vi "Generate SQL.vi"(8 "error in (no error)":errorcluster, 11 "SQLite Connection in":refnum<class "Connection.lvclass">) -> (0 "error out":errorcluster, 2 ".sql File Path":path, 3 "SQLite Connection out":refnum<class "Connection.lvclass">)   [LabVIEW 2024, in "DBMigrations.lvlib"]
doc: "Output schema and data to .sql file in same location as database."
uses:
  DBMigrations.lvlib
  <vilib>/drjdpowell/SQLite Library/SQL Connection/Connection.lvclass
  <vilib>/drjdpowell/SQLite Library/SQL Connection/Connection.lvclass/Connection.ctl
  <vilib>/Utility/error.llb/Trim Whitespace One-Sided.vi
  <vilib>/drjdpowell/SQLite Library/SQL Connection/Execute SQL (1D String).vi
  <vilib>/drjdpowell/SQLite Library/SQL Connection/Execute SQL.vi
  <vilib>/drjdpowell/SQLite Library/SQLite.lvlib
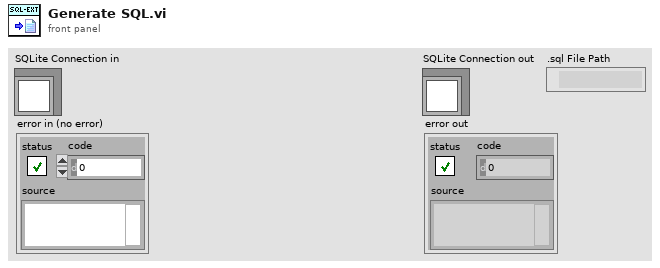
[diagram p1: front panel]
types:
  T1 = enum16{"open", "replace", "create", "open or create", "replace or create", "replace or create with confirmation"}
  T2 = typedef "DB-Migrations.lvlib/Schema.ctl" = cluster{"table name":string, "table info":cluster{"cid":string, "name":string, "type":string, "notnull":string, "dflt_value":string, "pk":string, "unique":string}[]}[]
  T3 = cluster{"cid":string, "name":string, "type":string, "notnull":string, "dflt_value":string, "pk":string, "unique":string}[]
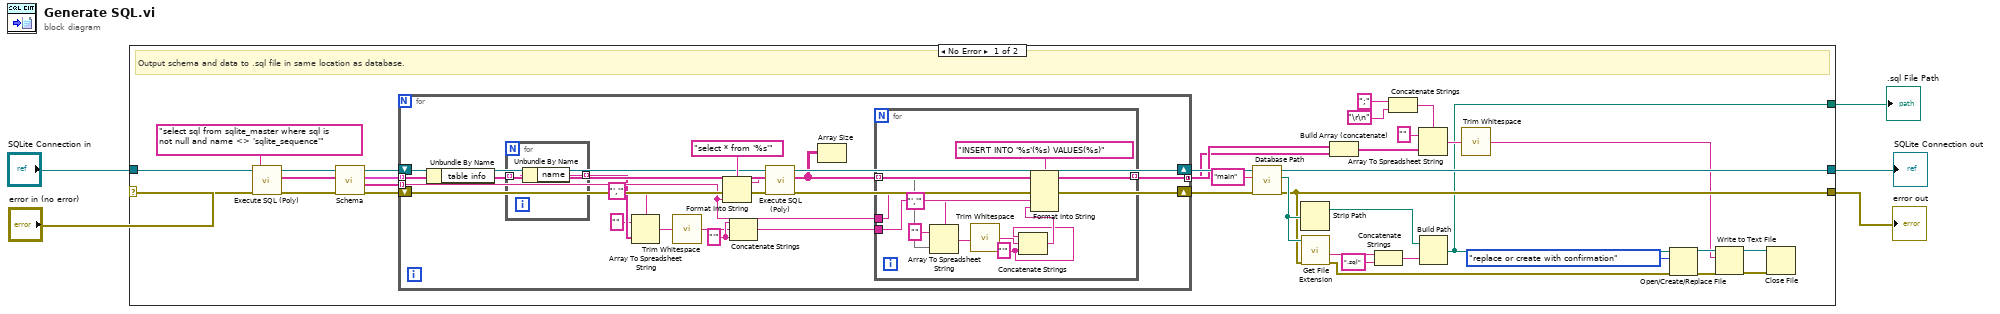
[diagram p0: block diagram]
diagram:
  n1 = case shown="No Error" "error in (no error)" {
    selector: "error in (no error)" -> [w22 w73]
    tunnel: "SQLite Connection in" -> [w40 w74]
    tunnel: [w37 w74] -> w4
    tunnel: [w29 w73] -> w3
    tunnel: [w21 _] -> w1
    frame No Error {
      # "Output schema and data to .sql file in same location as database."
      n2 = call-poly <vilib>:"Execute SQL (Poly).vi"("error in (no error)"=w22, "SQL"="select sql from sqlite_master where sql is not null and name <> 'sqlite_sequence'", "SQLite Connection in"=w40) -> ("error out"=w16:errorcluster, "Result Set"=w9:string[], "SQLite Connection"=w17:refnum<class "Connection.lvclass">)  [unwired: 5 in, 1 out]
      n3 = call "Schema.vi"("error in (no error)"=w16, "SQLite Connection In"=w17) -> ("error out"=w14:errorcluster, "Table Names"=w15:string[], "Schema"=w10:T2, "SQLite Connection Out"=w13:refnum<class "Connection.lvclass">)  [unwired: 6 in]
      n4 = for {
        tunnel: w15 -> [w49] mode=indexing
        shift-right: [w55] -> w12
        shift-left: w14 -> [w56]
        shift-right: [w53] -> w11
        shift-left: w13 -> [w54]
        tunnel: w10 -> [w51] mode=indexing
        tunnel: [w42] -> w7 mode=concatenating
        w43 = "'" ("string")
        n5 = Unbundle By Name(w51) -> ("table info"=w50:T3)
        n6 = for {
          tunnel: w50 -> [w61] mode=indexing
          tunnel: [w60] -> w48 mode=indexing
          n7 = Unbundle By Name(w61) -> ("name"=w60:string)
        }
        n8 = Array To Spreadsheet String(delimiter (Tab)="','", array=w48, 3:"" ("format string")) -> (spreadsheet string=w45:string)
        n9 = call <vilib>:"Trim Whitespace.vi"("string"=w45) -> ("trimmed string"=w41:string)  [unwired: 1 in]
        n10 = Format Into String(format string="select * from '%s'" ("SQL"), error in=w56, w49) -> (resulting string=w57:string, error out=w58:errorcluster)  [unwired: 1 in]
        n11 = Concatenate Strings(w43, w41, w43) -> (w44:string)
        n12 = call-poly <vilib>:"Execute SQL (Poly).vi"("error in (no error)"=w58, "SQL"=w57, "SQLite Connection in"=w54) -> ("error out"=w55:errorcluster, "Result Set"=w52:string[][], "SQLite Connection"=w53:refnum<class "Connection.lvclass">)  [unwired: 5 in, 1 out]
        n13 = Array Size(array=w52) -> ()  [unwired: 1 out]
        n14 = for {
          tunnel: w52 -> [w69] mode=indexing
          tunnel: w49 -> [w71]
          tunnel: w44 -> [w70]
          tunnel: [w63] -> w42 mode=indexing
          w64 = "'" ("string")
          n15 = Array To Spreadsheet String(delimiter (Tab)="','", array=w69, 3:"" ("format string")) -> (spreadsheet string=w65:string)
          n16 = call <vilib>:"Trim Whitespace.vi"("string"=w65) -> ("trimmed string"=w62:string)  [unwired: 1 in]
          n17 = Concatenate Strings(w64, w62, w64) -> (w66:string)
          n18 = Format Into String(format string="INSERT INTO '%s'(%s) VALUES(%s)" ("SQL"), w71, w70, w66) -> (resulting string=w63:string)  [unwired: 2 in, 1 out]
        }
      }
      n19 = call <vilib>:"Database Path.vi"("error in (no error)"=w12, "Database Name (\"main\")"="main" ("Database Name (\"main\")"), "SQLite Connection in"=w11) -> ("error out"=w29:errorcluster, "Path to Database"=w35:path, "SQLite Connection"=w37:refnum<class "Connection.lvclass">)  [unwired: 6 in]
      n20 = Strip Path(path=w35) -> (stripped path=w36:path)  [unwired: 1 out]
      n21 = call <vilib>:"Get File Extension.vi"("error in (no error)"=w29, "file"=w35) -> ("error out"=w30:errorcluster, "filename without extension"=w34:string)  [unwired: 5 in, 3 out]
      n22 = Build Array (concatenate)(w9, w7) -> (w8:string[])
      n23 = Concatenate Strings(w34, ".sql" ("string")) -> (w32:string)
      n24 = Concatenate Strings(";" ("delimiter (Tab)"), "\r\n") -> (w18:string)
      n25 = Array To Spreadsheet String(delimiter (Tab)=w18, array=w8, 3:"" ("format string")) -> (spreadsheet string=w25:string)
      n26 = Build Path(base path=w36, name or relative path=w32) -> (appended path=w21:path)
      n27 = call <vilib>:"Trim Whitespace.vi"("string"=w25) -> ("trimmed string"=w6:string)  [unwired: 1 in]
      n28 = Open/Create/Replace File(file path (use dialog)=w21, error in=w30, operation (0:open)=T1."replace or create with confirmation") -> (refnum out=w27:refnum<file>, error out=w26:errorcluster)  [unwired: 3 in, 1 out]
      n29 = Write to Text File(file (use dialog)=w27, text=w6, error in=w26) -> (refnum out=w24:refnum<file>, error out=w23:errorcluster)  [unwired: 1 in, 1 out]
      n30 = Close File(refnum=w24, error in=w23) -> ()  [unwired: 2 out]
    }
    frame Error {
    }
  }
  "SQLite Connection out" <- w4
  "error out" <- w3
  ".sql File Path" <- w1
